vi "HMI State Machine.vi"(7 "Get/Set State":T1, 9 "error in (no error)":errorcluster) -> (8 "State":T1, 10 "error out":errorcluster)   [LabVIEW 2019]
uses:
  HMI-States.ctl
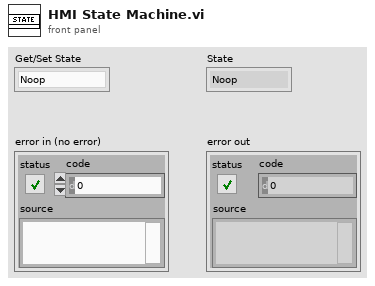
[diagram p1: front panel]
types:
  T1 = typedef "HMI-States.ctl" = enum16{"Noop", "Initialize", "Connect", "Reconnect", "Subscribe", "Publish", "Unsubscribe", "Disconnect", "Exit", "8", "9", "10", "11", "12", "13", "14", "15", "16", "17", "18", "19", "Idle", "Connected"}
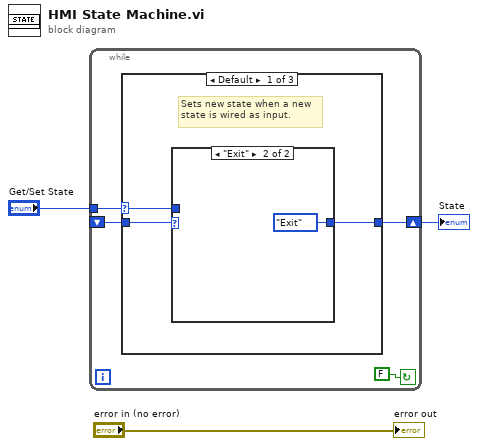
[diagram p0: block diagram]
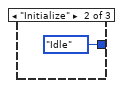
[diagram p3: hidden frame]
diagram:
  n1 = while {
    tunnel: "Get/Set State" -> [w7]
    shift-right: [w5] -> w2
    shift-left: _ -> [w6]
    stop <- FALSE continue-if-true
    n2 = case shown="Default" w7 {
      selector: w7 -> [w8 _ _]
      tunnel: [w9 HMI-States."Idle" ("Get/Set State") w14] -> w5
      tunnel: w6 -> [w10 _ w14]
      frame Default {
        # "Sets new state when a new\nstate is wired as input."
        n3 = case shown="\"Exit\"" w10 {
          tunnel: [w11 HMI-States."Exit" ("Get/Set State")] -> w9
          tunnel: w8 -> [w11 _]
          frame Default {
          }
          frame "Exit" {
          }
        }
      }
      frame "Initialize" {
      }
      frame "Noop" {
        # "Returns current state when\nno state is wired to input."
      }
    }
  }
  "State" <- w2
  "error out" <- "error in (no error)"
